vi "gmap_example_NO_hardware.vi"() -> ()   [LabVIEW 2025]
uses:
  <vilib>/sklein/WebView2 XControl/WebView2 XControl/WebView2 Control.xctl
panel:
  out "Map file":string=".html"
  in  "Route altitude, feet":dbl
  in  "Route speed, mph":dbl
  out "Coordinates":string
  in  "Send route":bool
  out "WebView2 Browser Control":string(xcontrol)
  in  "Refresh map":bool
  out "Status":string
  in  "stop":bool
  # "GNSS Simulation System (GPS Constellation)"
  # "Route options"
  # "System status"
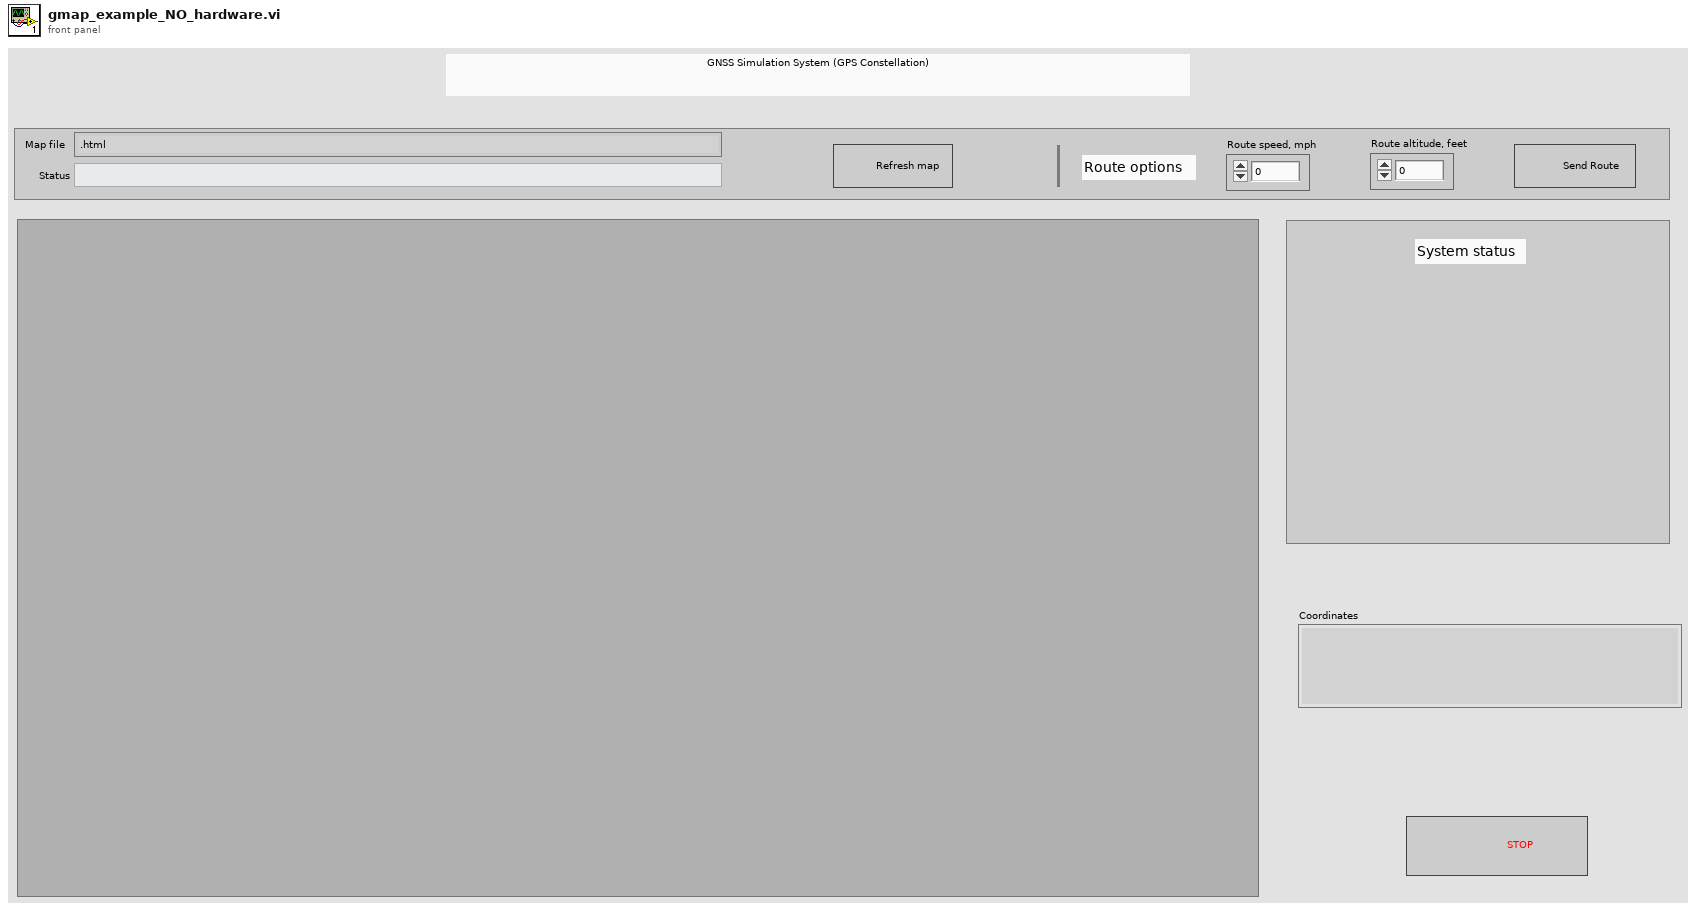
[diagram p1: front panel]
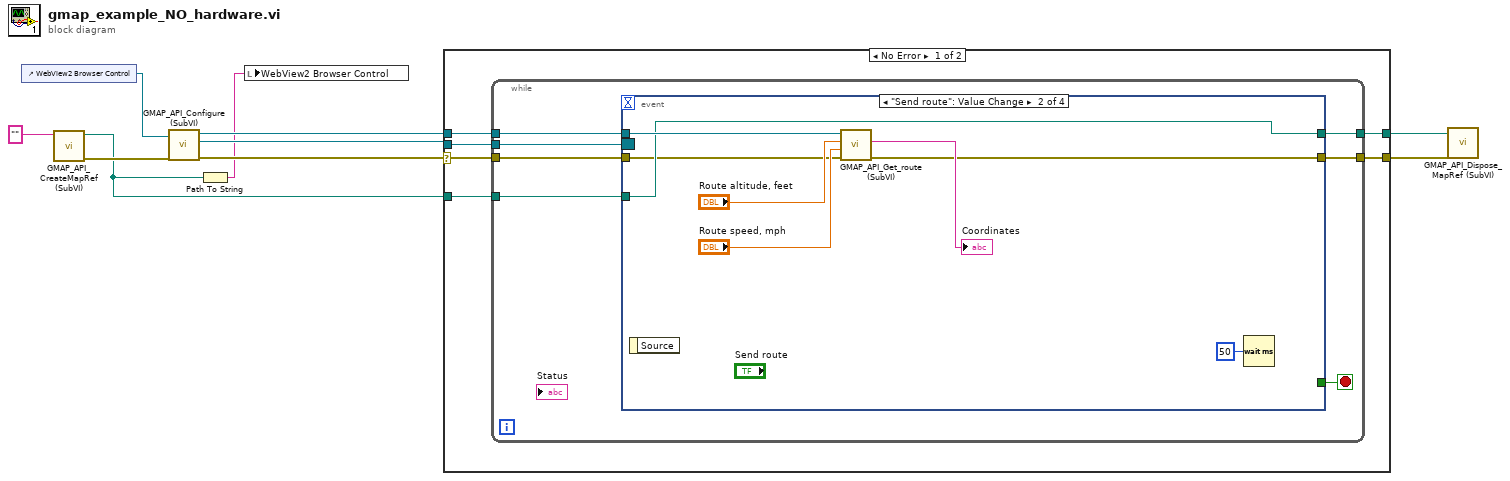
[diagram p0: block diagram]
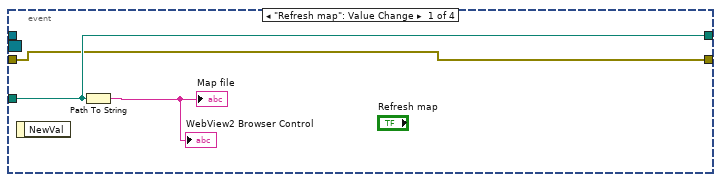
[diagram p2: hidden frame]
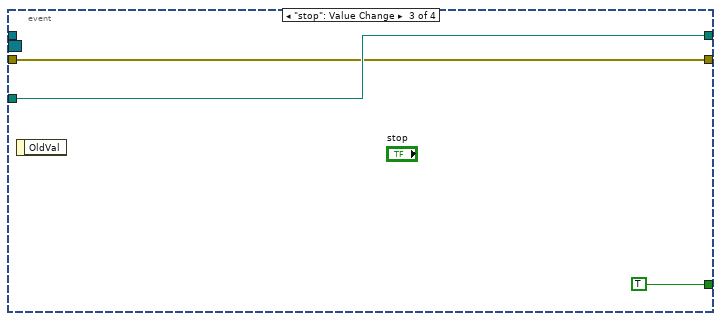
[diagram p3: hidden frame]
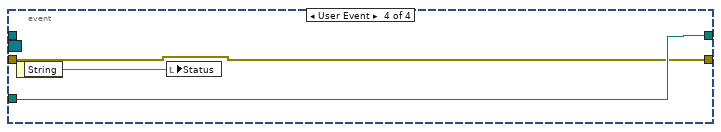
[diagram p4: hidden frame]
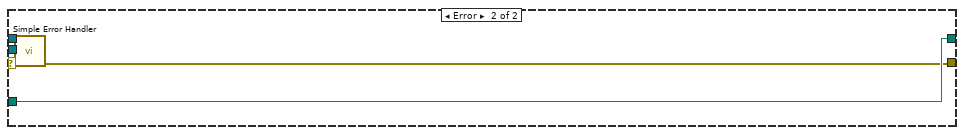
[diagram p5: hidden frame]
diagram:
  n1 = control-ref of="WebView2 Browser Control"() -> (w7:refnum<vi>)
  n2 = call "GMAP_API_CreateMapRef (SubVI).vi"("Gmaps API key"="") -> ("error out"=w5:errorcluster, "map file path"=w1:path)  [unwired: 9 in]
  n3 = call "GMAP_API_Configure (SubVI).vi"("error in"=w5, "Browser control in"=w7) -> ("error out"=w9:errorcluster, "Event Registration Refnum"=w10:refnum<event-registration>, "Browser control out"=w8:refnum<vi>)  [unwired: 7 in]
  n4 = Path To String(path=w1) -> (string=w2:string)
  n5 = local write "WebView2 Browser Control"(w2) -> ()
  n6 = case shown="No Error" w9 {
    selector: w9 -> [w12 w43]
    tunnel: w10 -> [w16 _]
    tunnel: w8 -> [w15 _]
    tunnel: w1 -> [w14 w42]
    tunnel: [w13 w42] -> w4
    tunnel: [w11 w41] -> w3
    frame No Error {
      n7 = while {
        tunnel: w16 -> [w23]
        tunnel: w15 -> [w21]
        tunnel: w14 -> [w20]
        tunnel: [w19] -> w13
        tunnel: w12 -> [w18]
        tunnel: [w17] -> w11
        stop <- w22 stop-if-true
        n8 = event shown="[1] \"Send route\": Value Change" {
          selector: w23 -> [_ _ _ _]
          dyn-events: _ -> [_ _ _ _]
          timeout: _ -> [_ _ _ _]
          tunnel: [_ _ TRUE _] -> w22
          tunnel: w21 -> [_ w34 _ _]
          tunnel: w20 -> [w26 w29 w36 w39]
          tunnel: [w26 w29 w36 w39] -> w19
          tunnel: w18 -> [w24 w28 w35 w38]
          tunnel: [w24 w27 w35 w38] -> w17
          event "Refresh map": Value Change {
            n9 = event-data() -> ()  [unwired: 1 in, 1 out]
            n10 = Path To String(path=w26) -> (string=→"WebView2 Browser Control" →"Map file":string)
          }
          event "Send route": Value Change {
            n11 = event-data() -> ()  [unwired: 1 in, 1 out]
            n12 = call "GMAP_API_Get_route (SubVI).vi"("error in (no error)"=w28, "Route speed, mph"="Route speed, mph", "Route altitude, feet"="Route altitude, feet", "Browser control ref in"=w34) -> ("error out"=w27:errorcluster, "Coordinates"=→"Coordinates":string)  [unwired: 4 in, 2 out]
            n13 = Wait (ms)(milliseconds to wait=u32 50) -> ()  [unwired: 1 out]
          }
          event "stop": Value Change {
            n14 = event-data() -> ()  [unwired: 1 in, 1 out]
          }
          event User Event {
            n15 = event-data() -> ("String"=w40:string)  [unwired: 1 in]
            n16 = local write "Status"(w40) -> ()
          }
        }
      }
    }
    frame Error {
      n17 = call <vilib>:"Simple Error Handler.vi"("error in (no error)"=w43) -> ("error out"=w41:errorcluster)  [unwired: 4 in, 4 out]
    }
  }
  n18 = call "GMAP_API_Dispose_MapRef (SubVI).vi"("error in"=w3, "map file path"=w4) -> ()  [unwired: 9 in, 1 out]
